vi "Save Profi map.vi"(7 "Write":bool, 8 "error in":errorcluster, 10 "configuration file path":path, 11 "Tempratures":cluster{"Name":T1, "Profi":T2, "Unit":T3}[][](array[cluster])) -> (0 "error out":errorcluster, 3 "transposed array":cluster{"Name":T1, "Profi":T2, "Unit":T3}[][](array[cluster]))   [LabVIEW 2025]
uses:
  <vilib>/Utility/config.llb/NI_LVConfig.lvlib
  controls/Tempratures.ctl
  controls/Profi address.ctl
  <vilib>/Utility/config.llb/Read Key (String).vi
  controls/Unit Temp.ctl
  <vilib>/Utility/config.llb/Write Key (String).vi
panel:
  out "Array 4":string[](array[string])
  out "Array 3":string[](array[string])
  out "Array 2":cluster{"Sensor":T1, "Profi":T2}[](array[cluster])
  out "Array":cluster{"Sensor":T1, "Profi":T2}[][](array[cluster])
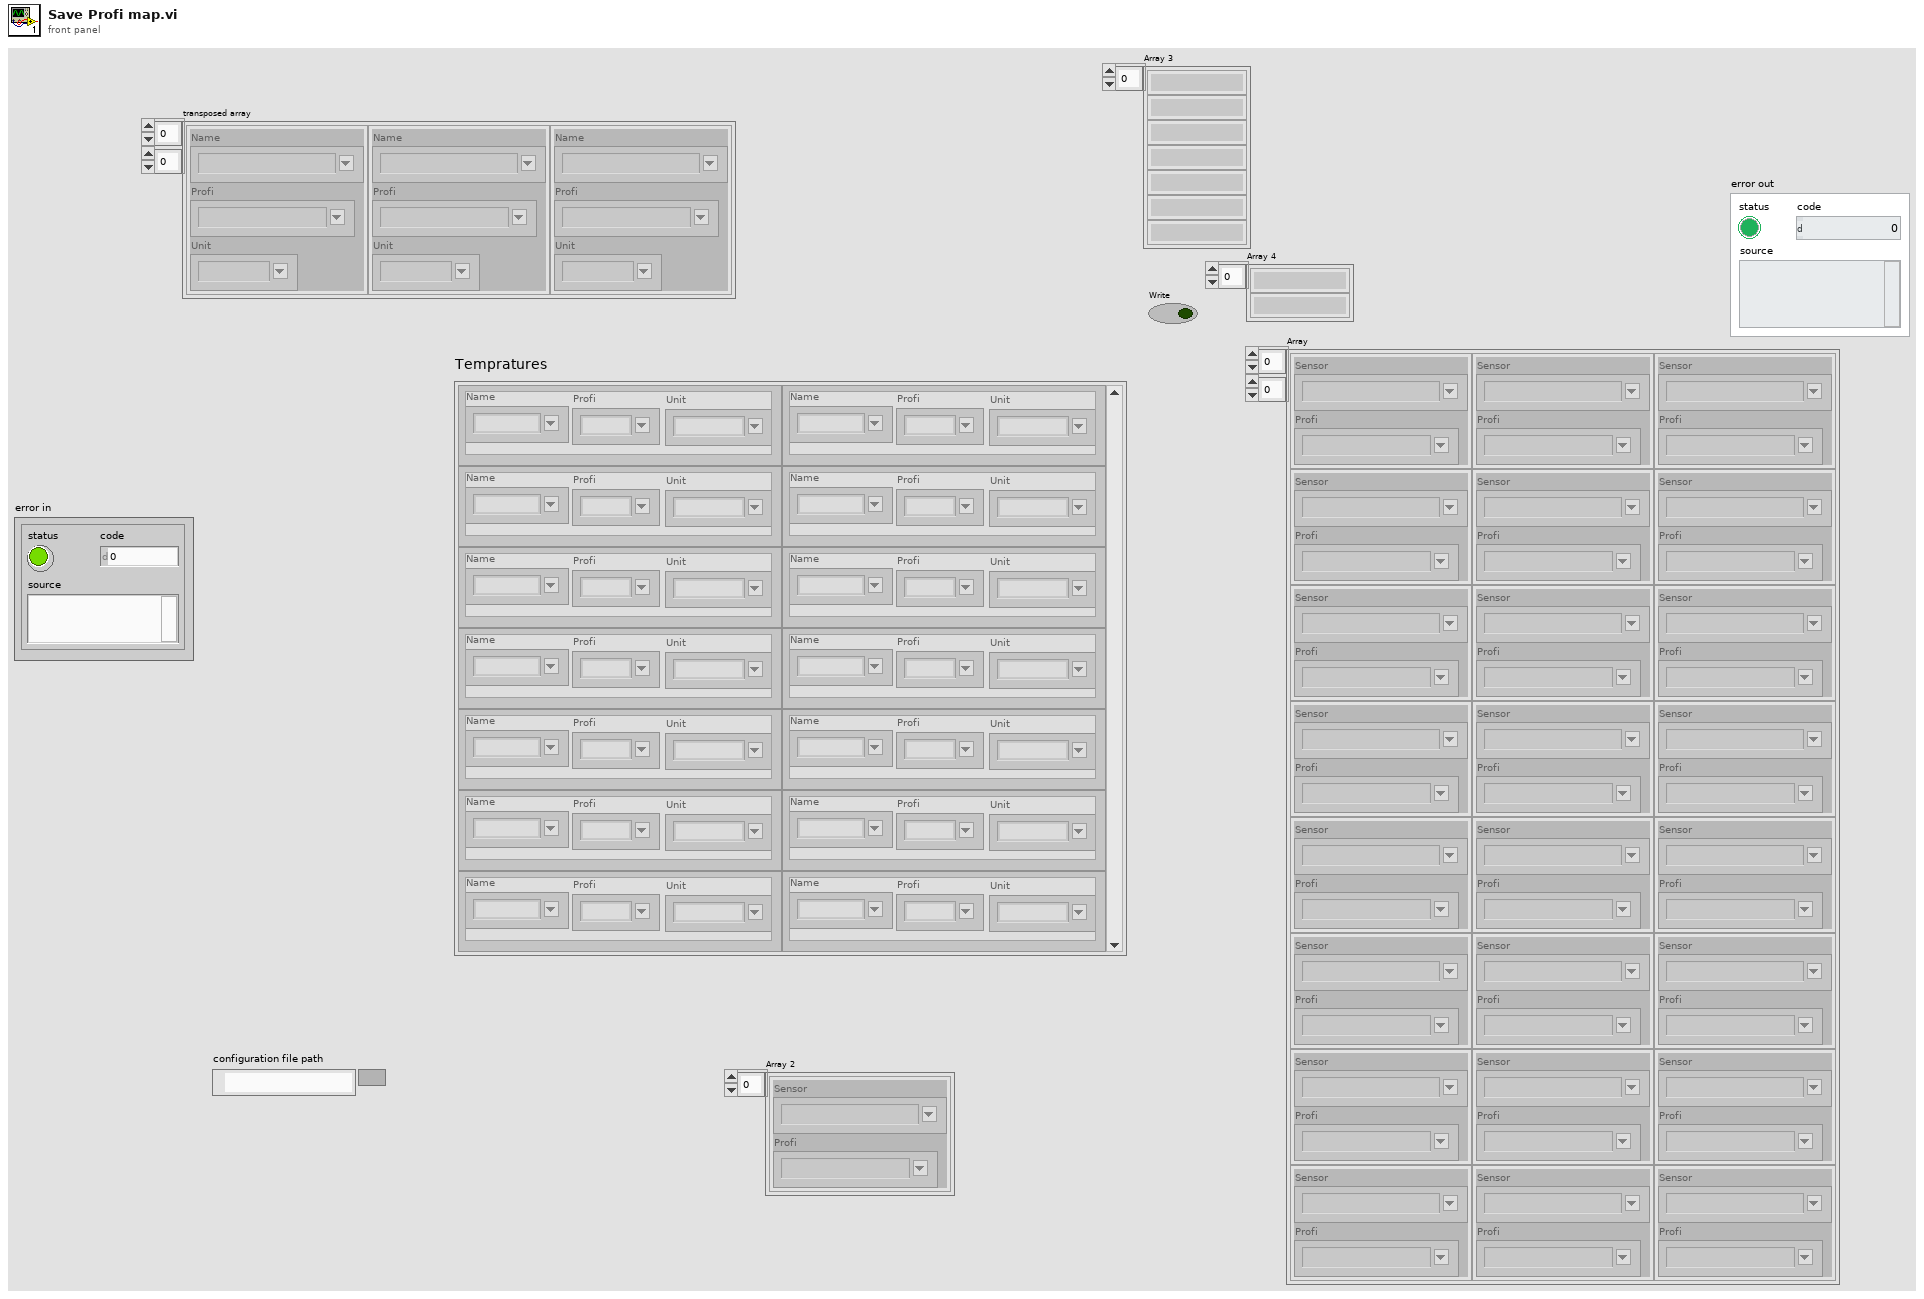
[diagram p1: front panel]
types:
  T1 = typedef "Tempratures.ctl" = string
  T2 = typedef "Profi address.ctl" = string
  T3 = typedef "Unit Temp.ctl" = string
  T4 = typedef "NI_LVConfig.lvlib/Config Data RefNum.ctl" = refnum<k1>
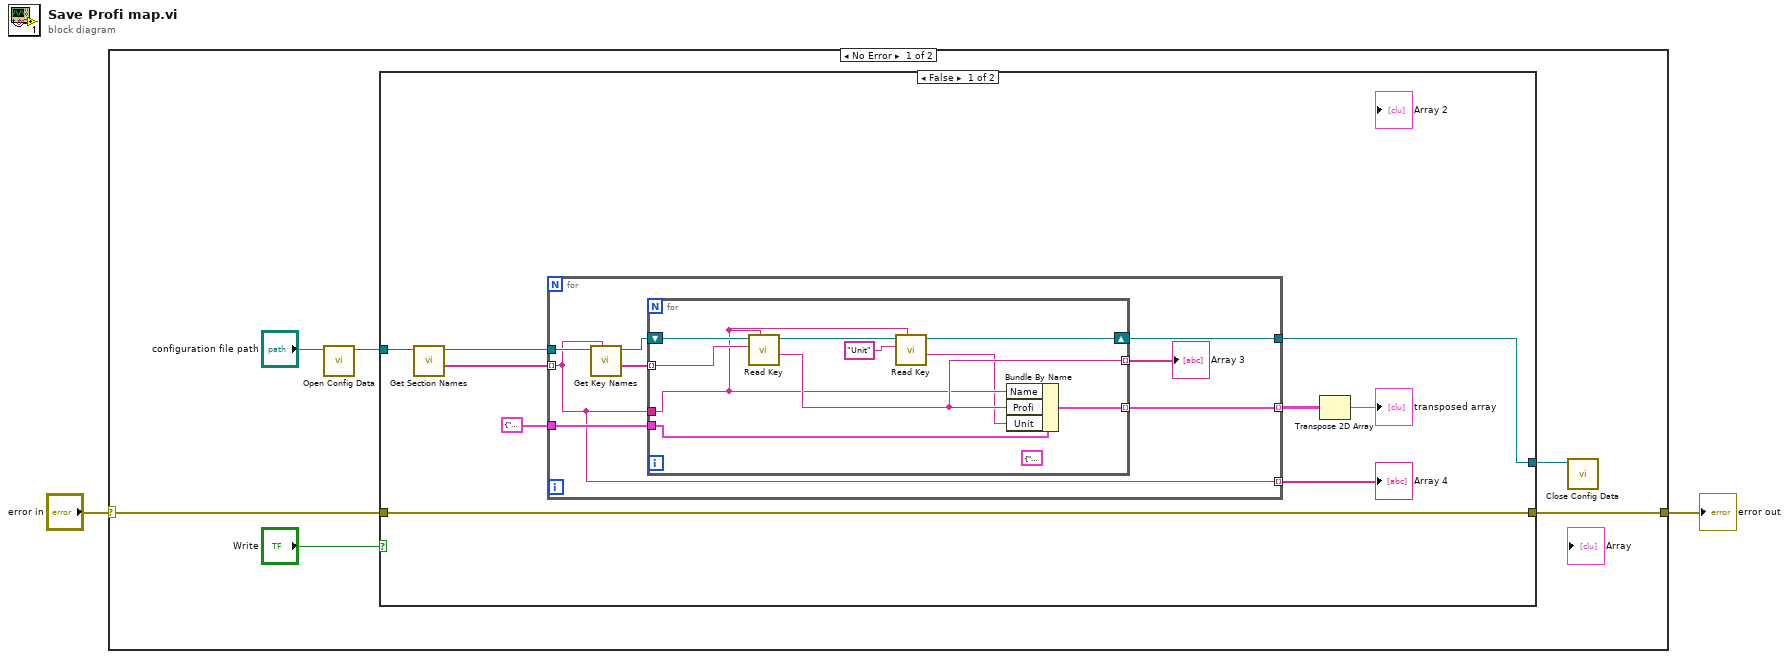
[diagram p0: block diagram]
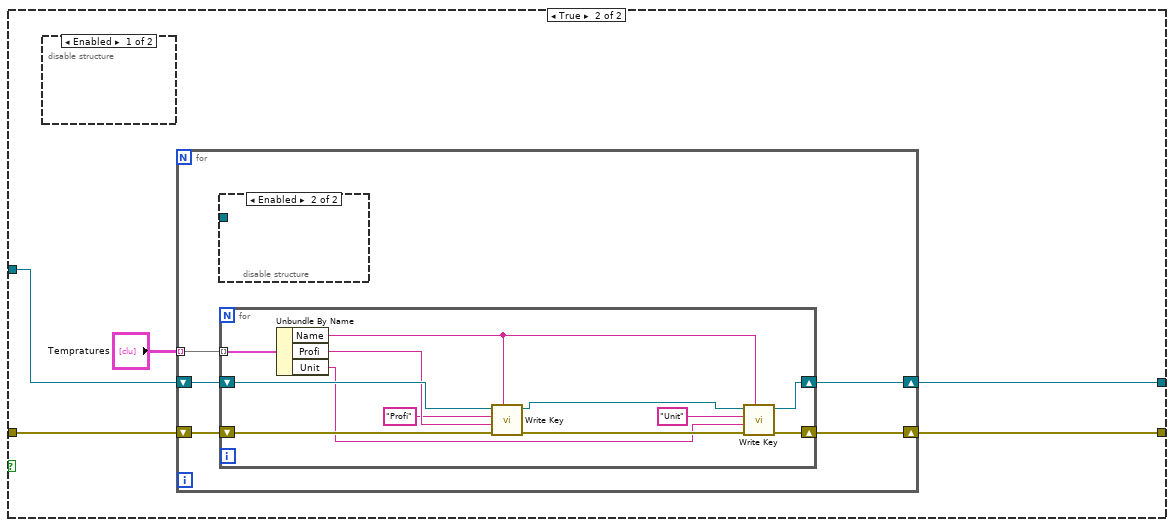
[diagram p2: hidden frame]
diagram:
  n1 = case shown="No Error" "error in" {
    selector: "error in" -> [w4 w59]
    tunnel: [w3 w59] -> w1
    frame No Error {
      n2 = call <vilib>:"Open Config Data.vi"("configuration file path"="configuration file path") -> ("refnum"=w8:T4)  [unwired: 8 in, 2 out]
      n3 = case shown="False" "Write" {
        tunnel: w8 -> [w16 w40]
        tunnel: [w17 w39] -> w5
        tunnel: w4 -> [w12 w38]
        tunnel: [w12 w37] -> w3
        frame False {
          n4 = call <vilib>:"Get Section Names.vi"("refnum"=w16) -> ("section names"=w15:string[], "refnum out"=w14:T4)  [unwired: 8 in, 1 out]
          n5 = for {
            tunnel: [w25] -> w17
            tunnel: w15 -> [w18] mode=indexing
            tunnel: w14 -> [w22]
            tunnel: [w21] -> w13 mode=indexing
            tunnel: cluster{"Name":T1, "Profi":T2, "Unit":T3} {"Name"="", "Profi"="", "Unit"=""} ("Cluster 6") -> [w19]
            tunnel: [w18] -> w9 mode=indexing
            n6 = call <vilib>:"Get Key Names.vi"("section"=w18, "refnum"=w22) -> ("key names"=w24:string[], "refnum out"=w23:T4)  [unwired: 6 in, 2 out]
            n7 = for {
              shift-right: [w29] -> w25
              shift-left: w23 -> [w35]
              tunnel: w24 -> [w33] mode=indexing
              tunnel: [w34] -> w21 mode=indexing
              tunnel: w18 -> [w28]
              tunnel: [w32] -> w20 mode=indexing
              tunnel: w19 -> [w31]
              (unwired) cluster{"Sensor":T1, "Profi":T2} {"Sensor"="", "Profi"=""} ("Cluster 6")
              n8 = call-poly <vilib>:"Read Key.vi"("section"=w28, "key"=w33, "refnum"=w35) -> ("value"=w32:string, "refnum out"=w30:T4)  [unwired: 5 in, 2 out]
              n9 = call-poly <vilib>:"Read Key.vi"("section"=w28, "key"="Unit", "refnum"=w30) -> ("value"=w26:string, "refnum out"=w29:T4)  [unwired: 5 in, 2 out]
              n10 = Bundle By Name(cluster=w31, "Name"=w28, "Profi"=w32, "Unit"=w26) -> (w34:cluster{"Name":T1, "Profi":T2, "Unit":T3})
            }
            "Array 3" <- w20
          }
          "Array 4" <- w9
          n11 = Transpose 2D Array(2D array=w13) -> (transposed array=→"transposed array":cluster{"Name":T1, "Profi":T2, "Unit":T3}[][])
        }
        frame True {
          n12 = disable-structure shown="Enabled" {
            frame Enabled {
            }
            frame Disabled {
            }
          }
          n13 = for {
            tunnel: "Tempratures" -> [w45] mode=indexing
            shift-right: [w43] -> w39
            shift-left: w40 -> [w44]
            shift-right: [w41] -> w37
            shift-left: w38 -> [w42]
            n14 = disable-structure shown="Enabled" {
              disable-tunnel: _ -> [w58 _]
              frame Disabled {
              }
              frame Enabled {
              }
            }
            n15 = for {
              tunnel: w45 -> [w57] mode=indexing
              shift-right: [w50] -> w43
              shift-left: w44 -> [w56]
              shift-right: [w51] -> w41
              shift-left: w42 -> [w54]
              n16 = Unbundle By Name(w57) -> ("Name"=w48:T1, "Profi"=w55:T2, "Unit"=w49:T3)
              n17 = call-poly <vilib>:"Write Key.vi"("section"=w48, "error in (no error)"=w54, "value"=w55, "key"="Profi", "refnum"=w56) -> ("error out"=w52:errorcluster, "refnum out"=w53:T4)  [unwired: 4 in, 1 out]
              n18 = call-poly <vilib>:"Write Key.vi"("section"=w48, "error in (no error)"=w52, "value"=w49, "key"="Unit", "refnum"=w53) -> ("error out"=w51:errorcluster, "refnum out"=w50:T4)  [unwired: 4 in, 1 out]
            }
          }
        }
      }
      n19 = call <vilib>:"Close Config Data.vi"("refnum"=w5) -> ()  [unwired: 9 in, 2 out]
    }
    frame Error {
    }
  }
  "error out" <- w1
